vi "LVA Session.vi"() -> ()   [LabVIEW 2020]
uses:
  scripting-server/Scripting Server/open_vi Argument--cluster.ctl
  scripting-server/Scripting Server/open_vi (Reply Payload)--cluster.ctl
  scripting-server/Scripting Server/save_vi Argument--cluster.ctl
  scripting-server/Scripting Server/save_vi (Reply Payload)--cluster.ctl
  scripting-server/Scripting Server/LVA_State.vi
  scripting-server/Scripting Server/Do Save VI.vi
  gateway/Error_to_string.vi
  scripting-server/Scripting Server/Do Open Vi.vi
  scripting-server/Scripting Server/Scripting Server.lvlib
panel:
  in  "ArgSave":T1
  in  "ArgOpen":T2
  in  "Tool":string
  out "Iters":dbl
  out "ErrSave":string
  out "ReplySave":string
  out "ErrOpen":string
  out "ReplyOpen":string
  out "ErrSave":string
  out "ErrOpen":string
  out "ReplySave":string
  out "ReplyOpen":string
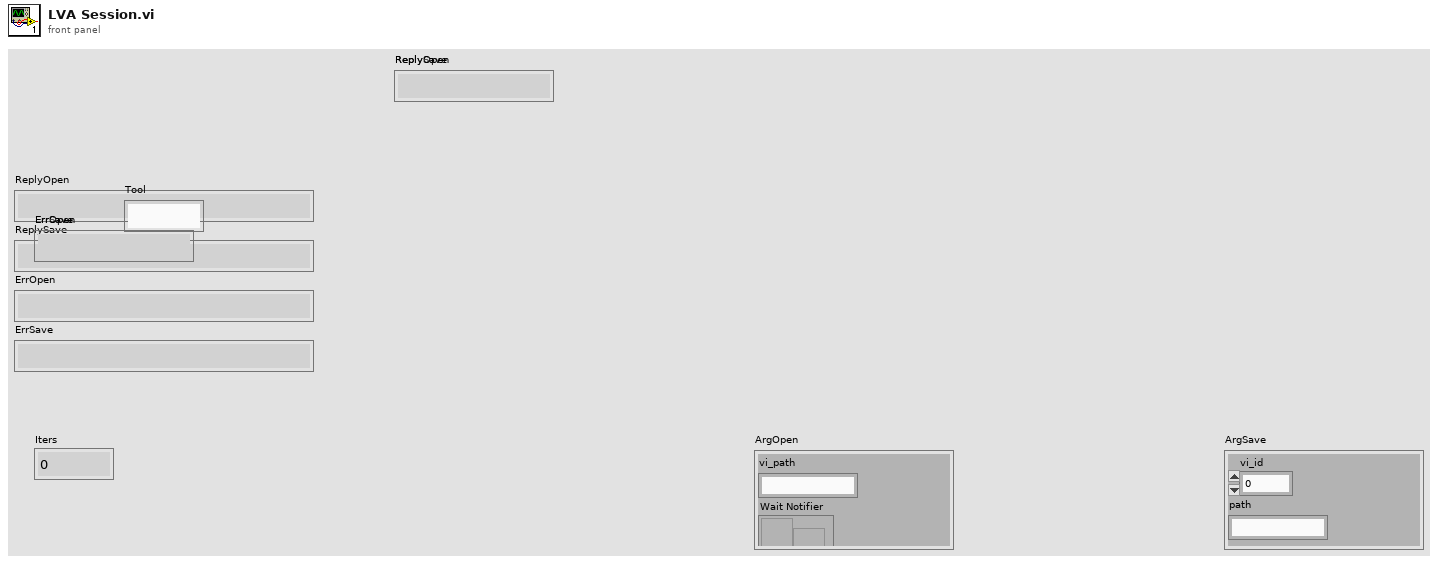
[diagram p1: front panel]
types:
  T1 = typedef "Scripting Server.lvlib/save_vi Argument--cluster.ctl" = cluster{"vi_id":i32, "path":string, "Wait Notifier":refnum<notifier>, "wait for reply":bool}
  T2 = typedef "Scripting Server.lvlib/open_vi Argument--cluster.ctl" = cluster{"vi_path":string, "Wait Notifier":refnum<notifier>, "wait for reply":bool}
  T3 = typedef "Scripting Server.lvlib/Module Data--cluster.ctl" = cluster{"Status":string, "Current ID":i32, "References":variant, "Config Data":T4, "MCP id":i32, "Log":string}
  T4 = typedef "Scripting Server.lvlib/Config Data.ctl" = cluster{"Allowed Paths":string[]}
  T5 = typedef "Scripting Server.lvlib/open_vi (Reply Payload)--cluster.ctl" = cluster{"vi_id":string, "error":errorcluster}
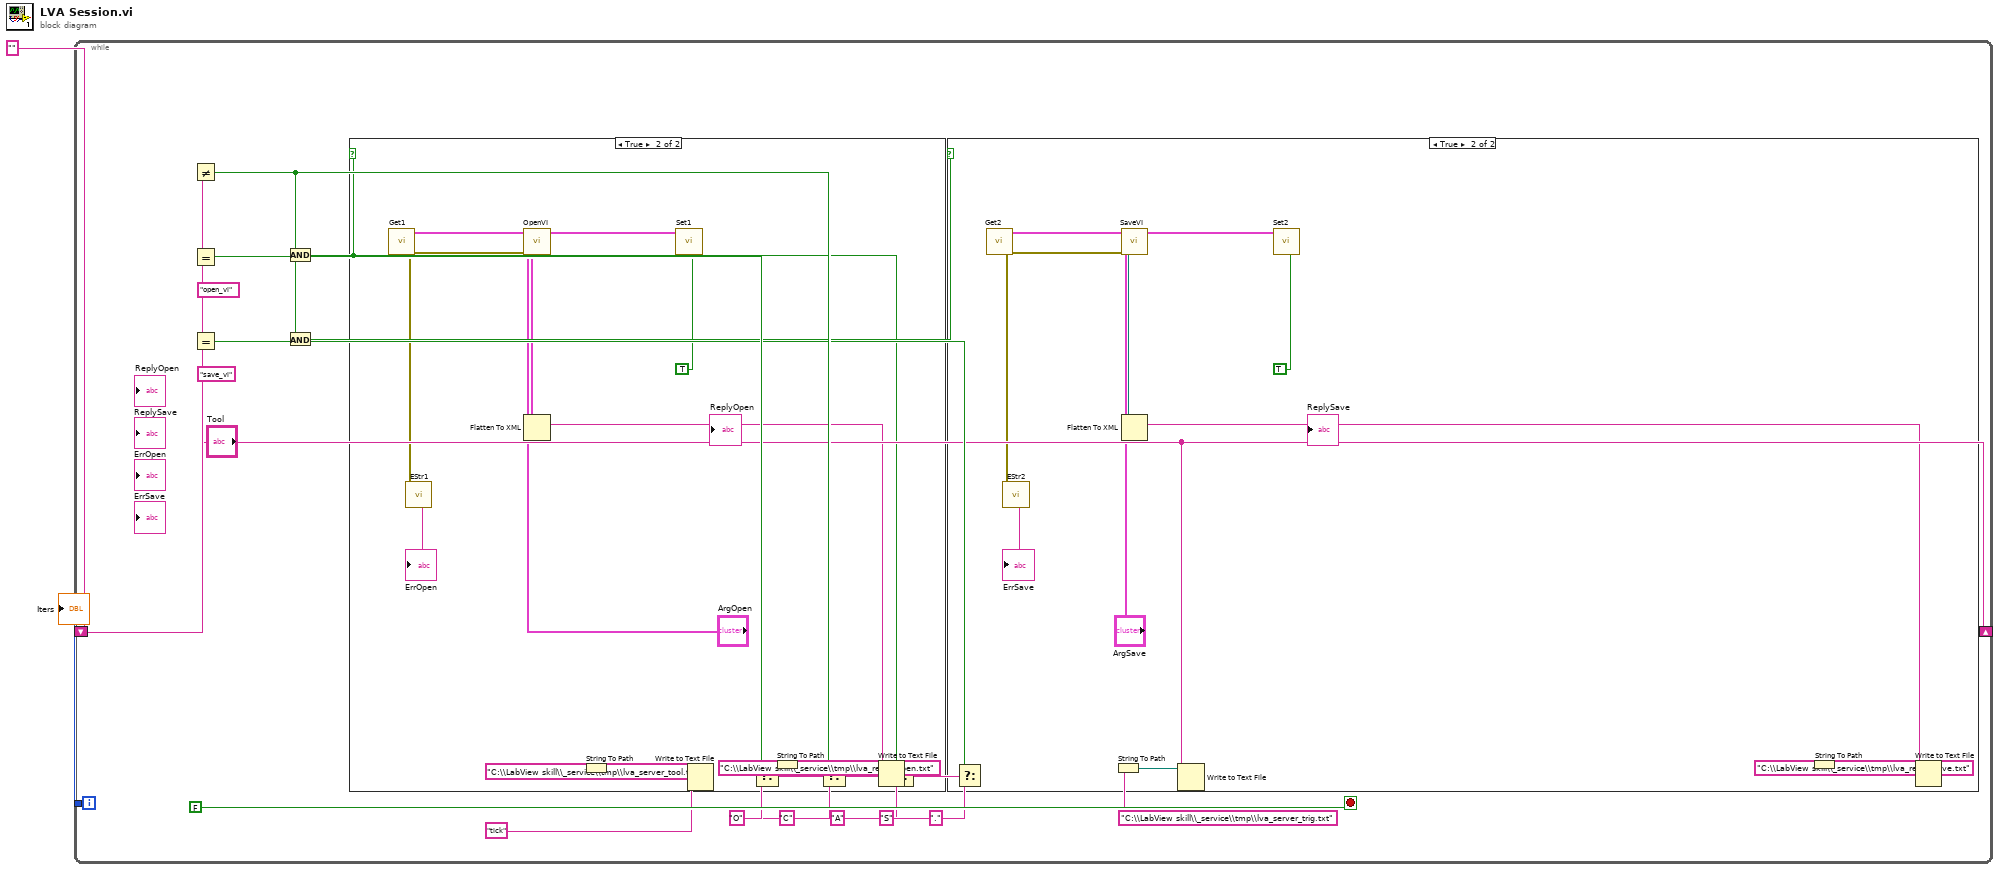
[diagram p0: block diagram]
diagram:
  n1 = while "Loop1" {
    shift-right: ["Tool"] -> _
    shift-left: "" ("SRInit") -> [w20]
    tunnel: [w18] -> w1
    i -> [w18]
    stop <- FALSE ("NeverStop") stop-if-true
    n2 = Not Equal? ("Chg")(x=w20, y="Tool") -> (x != y?=w22:bool)
    n3 = Equal? ("Eq1")(x="Tool", y="open_vi" ("SC1")) -> (x = y?=w23:bool)
    n4 = Equal? ("Eq2")(x="Tool", y="save_vi" ("SC2")) -> (x = y?=w21:bool)
    n5 = And ("And1")(x=w23, y=w22) -> (x .and. y?=w3:bool)
    n6 = And ("And2")(x=w21, y=w22) -> (x .and. y?=w19:bool)
    n7 = case "Case1" shown="True" w3 {
      frame False {
      }
      frame True {
        n8 = call "Get1"() -> ("Data Cluster"=w46:T3)  [unwired: 10 in, 1 out]
        n9 = call "OpenVI"("open_vi Argument"="ArgOpen", "Data Cluster in"=w46) -> ("error out"=w41:errorcluster, "open_vi (Reply Payload)"=w43:T5, "Data Cluster out"=w45:T3)  [unwired: 7 in]
        n10 = call "EStr1"("error in (no error)"=w41) -> ("spreadsheet string out"=→"ErrOpen":string)  [unwired: 10 in]
        n11 = Flatten To XML ("XML1")(6:w43) -> (2:w42:string)
        "ReplyOpen" <- w42
        n12 = call "Set1"("SetDC"=TRUE ("SetT1"), "Data Cluster 2"=w45) -> ()  [unwired: 8 in, 2 out]
        n13 = String To Path ("S2P1")(string="C:\\LabView skill\\_service\\tmp\\lva_reply_open.txt" ("PathOpen")) -> (path=w38:path)
        n14 = Write to Text File ("WT1")(file (use dialog)=w38, text=w42) -> ()  [unwired: 2 in, 3 out]
      }
    }
    n15 = String To Path ("S2P3")(string="C:\\LabView skill\\_service\\tmp\\lva_server_tool.txt" ("PT3")) -> (path=w16:path)
    n16 = Write to Text File ("WT3")(file (use dialog)=w16, text="tick" ("TICK")) -> ()  [unwired: 2 in, 3 out]
    n17 = Select ("SEL_E")(t="O" ("TE"), s=w23, f="." ("DOT")) -> (s? t:f=w7:string)
    n18 = Select ("SEL_C")(t="C" ("TC"), s=w22, f=w7) -> (s? t:f=w6:string)
    n19 = Select ("SEL_A")(t="A" ("TA"), s=w3, f=w6) -> (s? t:f=w5:string)
    n20 = case "Case2" shown="True" w19 {
      frame False {
      }
      frame True {
        n21 = call "Get2"() -> ("Data Cluster"=w36:T3)  [unwired: 10 in, 1 out]
        n22 = call "SaveVI"("save_vi Argument"="ArgSave", "Data Cluster in"=w36) -> ("error out"=w31:errorcluster, "VI Path"=w33:path, "Data Cluster out"=w35:T3)  [unwired: 7 in]
        n23 = call "EStr2"("error in (no error)"=w31) -> ("spreadsheet string out"=→"ErrSave":string)  [unwired: 10 in]
        n24 = Flatten To XML ("XML2")(6:w33) -> (2:w32:string)
        "ReplySave" <- w32
        n25 = call "Set2"("SetDC"=TRUE ("SetT2"), "Data Cluster 2"=w35) -> ()  [unwired: 8 in, 2 out]
        n26 = String To Path ("S2P2")(string="C:\\LabView skill\\_service\\tmp\\lva_reply_save.txt" ("PathSave")) -> (path=w28:path)
        n27 = Write to Text File ("WT2")(file (use dialog)=w28, text=w32) -> ()  [unwired: 2 in, 3 out]
      }
    }
    n28 = Select ("SEL_S")(t="S" ("TS"), s=w21, f=w5) -> ()  [unwired: 1 out]
    n29 = String To Path ("S2P4")(string="C:\\LabView skill\\_service\\tmp\\lva_server_trig.txt" ("PF4")) -> (path=w9:path)
    n30 = Write to Text File ("WT4")(file (use dialog)=w9, text="Tool") -> ()  [unwired: 2 in, 3 out]
  }
  "Iters" <- w1
